vi "Host - Get Local and ECAT Masters With Retries.vi"(8 "error in (no error)":errorcluster, 11 "serverName":string) -> (0 "error out":errorcluster, 1 "Message output":string, 2 "All Local Mods":refnum<k21>[](array[refnum]), 3 "All ECAT Masters":refnum<k21>[](array[refnum]))   [LabVIEW 2020, in "SEECD System Explorer.lvlib"]
uses:
  SEECD System Explorer.lvlib
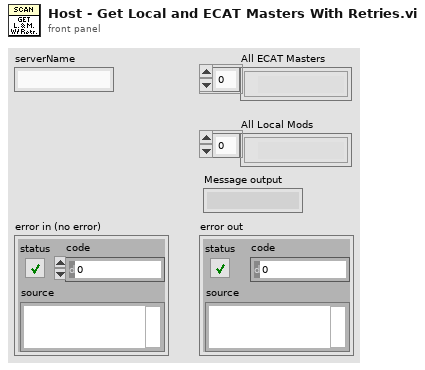
[diagram p1: front panel]
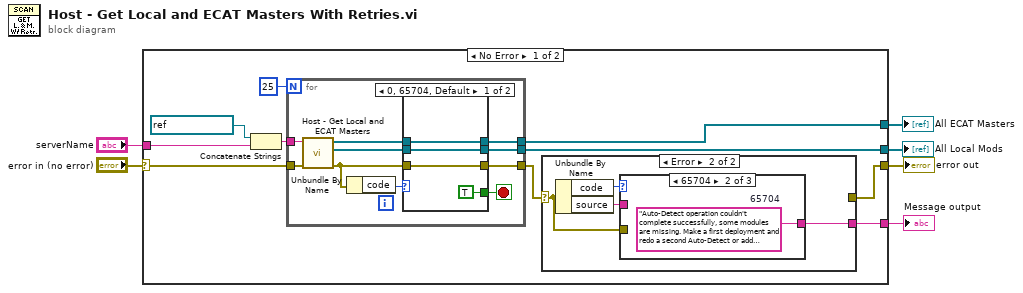
[diagram p0: block diagram]
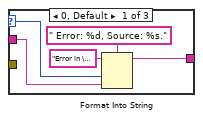
[diagram p3: hidden frame]
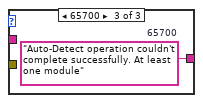
[diagram p4: hidden frame]
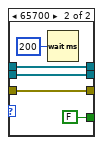
[diagram p5: hidden frame]
diagram:
  n1 = case shown="No Error" "error in (no error)" {
    selector: "error in (no error)" -> [w8 w48]
    tunnel: [w16 w48] -> w6
    tunnel: [w13 _] -> w5
    tunnel: [w11 _] -> w4
    tunnel: "serverName" -> [w10 _]
    tunnel: [w7 _] -> w1
    frame No Error {
      n2 = Concatenate Strings(refnum<k21> "ni.var.io://" ("IOV Engine in"), w10) -> (w12:string)
      n3 = for {
        N: 25 -> [_]
        tunnel: [w34] -> w11
        tunnel: w12 -> [w37]
        tunnel: [w32] -> w13
        tunnel: w8 -> [w38]
        tunnel: [w30] -> w15
        stop <- w29 stop-if-true
        n4 = call "Host - Get Local and ECAT Masters.vi"("error in (no error)"=w38, "Refnum in"=w37) -> ("error out"=w31:errorcluster, "All Local Mods"=w33:refnum<k21>[], "All ECAT Masters"=w35:refnum<k21>[])  [unwired: 6 in, 1 out]
        n5 = Unbundle By Name(w31) -> ("code"=w36:i32)
        n6 = case shown="0, 65704, Default" w36 {
          tunnel: w35 -> [w42 w47]
          tunnel: [w42 w47] -> w34
          tunnel: w33 -> [w41 w46]
          tunnel: [w41 w46] -> w32
          tunnel: w31 -> [w40 w44]
          tunnel: [w40 w44] -> w30
          tunnel: [TRUE FALSE] -> w29
          frame 0, 65704, Default {
          }
          frame 65700 {
            n7 = Wait (ms)(milliseconds to wait=u32 200) -> ()  [unwired: 1 out]
          }
        }
      }
      n8 = case shown="Error" w15 {
        selector: w15 -> [w17 w20]
        tunnel: [w17 _] -> w16
        tunnel: [_ w18] -> w7
        frame No Error {
        }
        frame Error {
          n9 = Unbundle By Name(w20) -> ("code"=w21:i32, "source"=w19:string)
          n10 = case shown="65704" w21 {
            selector: w21 -> [w24 _ _]
            tunnel: w20 -> [_ _ _]
            tunnel: [w22 w27 w28] -> w18
            tunnel: w19 -> [w23 _ _]
            frame 0, Default {
              n11 = Format Into String(format string=" Error: %d, Source: %s.", initial string="Error in \"Host - Get Local and ECAT Masters.vi\".", w24, w23) -> (resulting string=w22:string)  [unwired: 1 in, 1 out]
            }
            frame 65704 {
              w27 = "Auto-Detect operation couldn't complete successfully, some modules are missing. Make a first deployment and redo a second Auto-Detect or add manually missing local modules. "  # 65704
            }
            frame 65700 {
              w28 = "Auto-Detect operation couldn't complete successfully. At least one module"  # 65700
            }
          }
        }
      }
    }
    frame Error {
    }
  }
  "error out" <- w6
  "All Local Mods" <- w5
  "All ECAT Masters" <- w4
  "Message output" <- w1
